vi "to_json.vi"(8 "error in":errorcluster, 11 "mcap in":refnum<class "mcap.lvclass">) -> (0 "error out":errorcluster, 2 "json":string, 3 "mcap out":refnum<class "mcap.lvclass">, 4 "Not Default":bool)   [LabVIEW 2020, in "nominal types.lvlib" / "timestampManifest.lvlib" / "mcap.lvclass"]
uses:
  mcap.lvclass
  mcap.lvclass/mcap.ctl
  <vilib>/JDP Science/JSONtext/support/Format JSON Object.vi
  <vilib>/JDP Science/JSONtext/JSONtext.lvlib
  filterTypes/filterTypes.lvclass
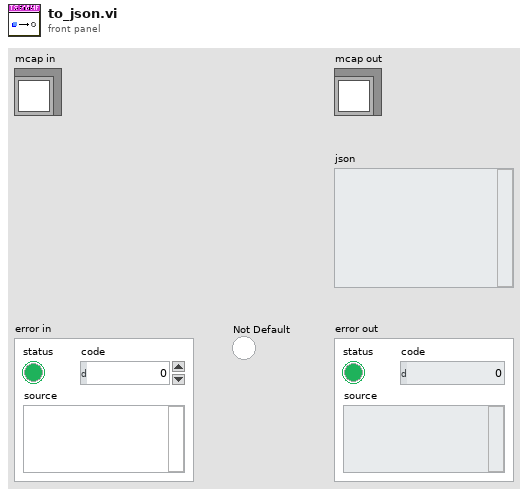
[diagram p1: front panel]
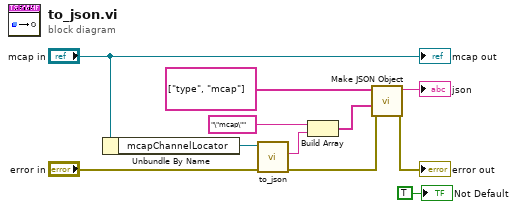
[diagram p0: block diagram]
diagram:
  n1 = Unbundle By Name("mcap in") -> ("mcapChannelLocator"=w10:refnum<class "filterTypes.lvclass">)
  n2 = call-dynamic "to_json.vi"("error in"="error in", "filterTypes in"=w10) -> ("error out"=w3:errorcluster, "json"=w8:string)  [unwired: 6 in, 2 out]
  n3 = Build Array("\"mcap\"" ("element"), w8) -> (w5:string[])
  n4 = call <vilib>:"Make JSON Object.vi"("error in (no error)"=w3, "JSON Items"=w5, "Item Names"=string[] ["type", "mcap"]) -> ("error out"=→"error out":errorcluster, "<JSON>"=→"json":string)  [unwired: 7 in]
  "mcap out" <- "mcap in"
  "Not Default" <- TRUE ("Not Default")
